vi "TEST_LvMarkdown.vi"() -> ()   [LabVIEW 2021]
uses:
  LvMarkdown/LineBreak/LineBreak.lvclass
  LvMarkdown/Heading/Heading.lvclass
  LvMarkdown/Collection/Collection.lvclass
  LvMarkdown/Paragraph/Paragraph.lvclass
  LvMarkdown/Line/Line.lvclass
  LvMarkdown/HorizontalRule/HorizontalRule.lvclass
  LvMarkdown/Code/Code.lvclass
  LvMarkdown/Bold/Bold.lvclass
  LvMarkdown/Italic/Italic.lvclass
  LvMarkdown/Strikethrough/Strikethrough.lvclass
  LvMarkdown/Blockquote/Blockquote.lvclass
  LvMarkdown/OrderedList/OrderedList.lvclass
  LvMarkdown/UnorderedList/UnorderedList.lvclass
  LvMarkdown/TaskList/TaskList.lvclass
  LvMarkdown/Image/Image.lvclass
  LvMarkdown/Url/Url.lvclass
  LvMarkdown/Link/Link.lvclass
  LvMarkdown/Table/Table.lvclass
  LvMarkdown/Alignment/Alignment.lvclass
  LvMarkdown/FencedCodeBlock/FencedCodeBlock.lvclass
  LvMarkdown/FootnoteReference/FootnoteReference.lvclass
  LvMarkdown/Footnote/Footnote.lvclass
  LvMarkdown/LinkingHeadingId/LinkingHeadingId.lvclass
  LvMarkdown/DefinitionList/DefinitionList.lvclass
  <vilib>/ErrorRing/Error Ring.xnode
  b2edfd4d-23ef-4285-98b5-6188740e71bd.vi
  TEST_LvMarkdownStep.ctl
  LvMarkdown/Alignment/AlignmentEnum.ctl
panel:
  out "String out":string
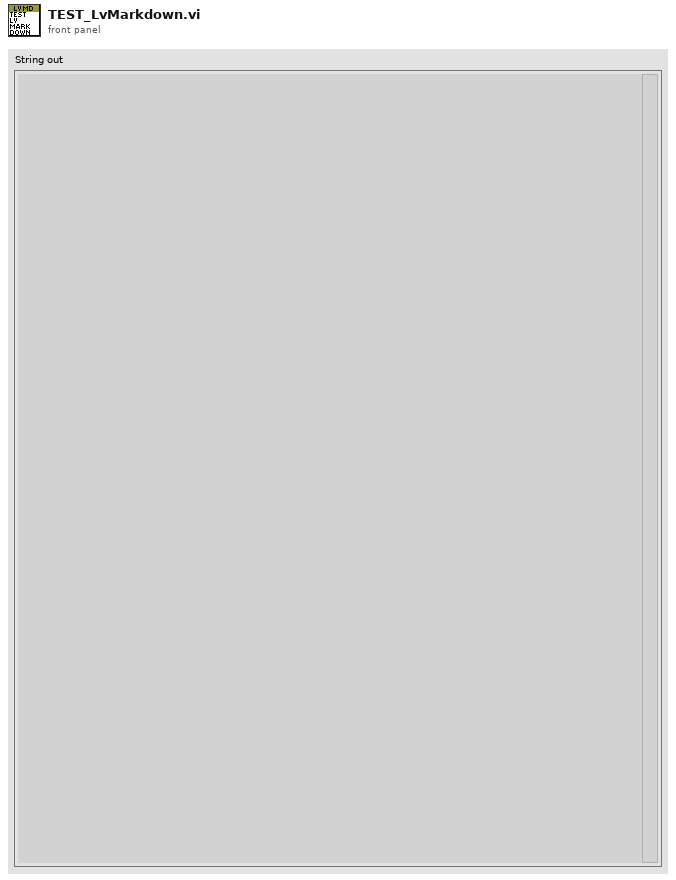
[diagram p1: front panel]
types:
  T1 = enum16{"Level 1", "Level 2", "Level 3", "Level 4", "Level 5", "Level 6"}
  T2 = typedef "TEST_LvMarkdownStep.ctl" = enum16{"Init", "Heading 1", "Paragraph 1", "Heading 2", "Paragraph 2", "Line", "Horizontal Rule", "Emphasis", "Blockquote", "List", "Image", "URL", "Link", "Table", "FencedCodeBlock", "Footnote", "LinkingHeadingId", "DefinitionList", "Exit"}
  T3 = typedef "LvMarkdown.lvlib/Alignment.lvclass/AlignmentEnum.ctl" = enum16{"Left", "Center", "Right"}
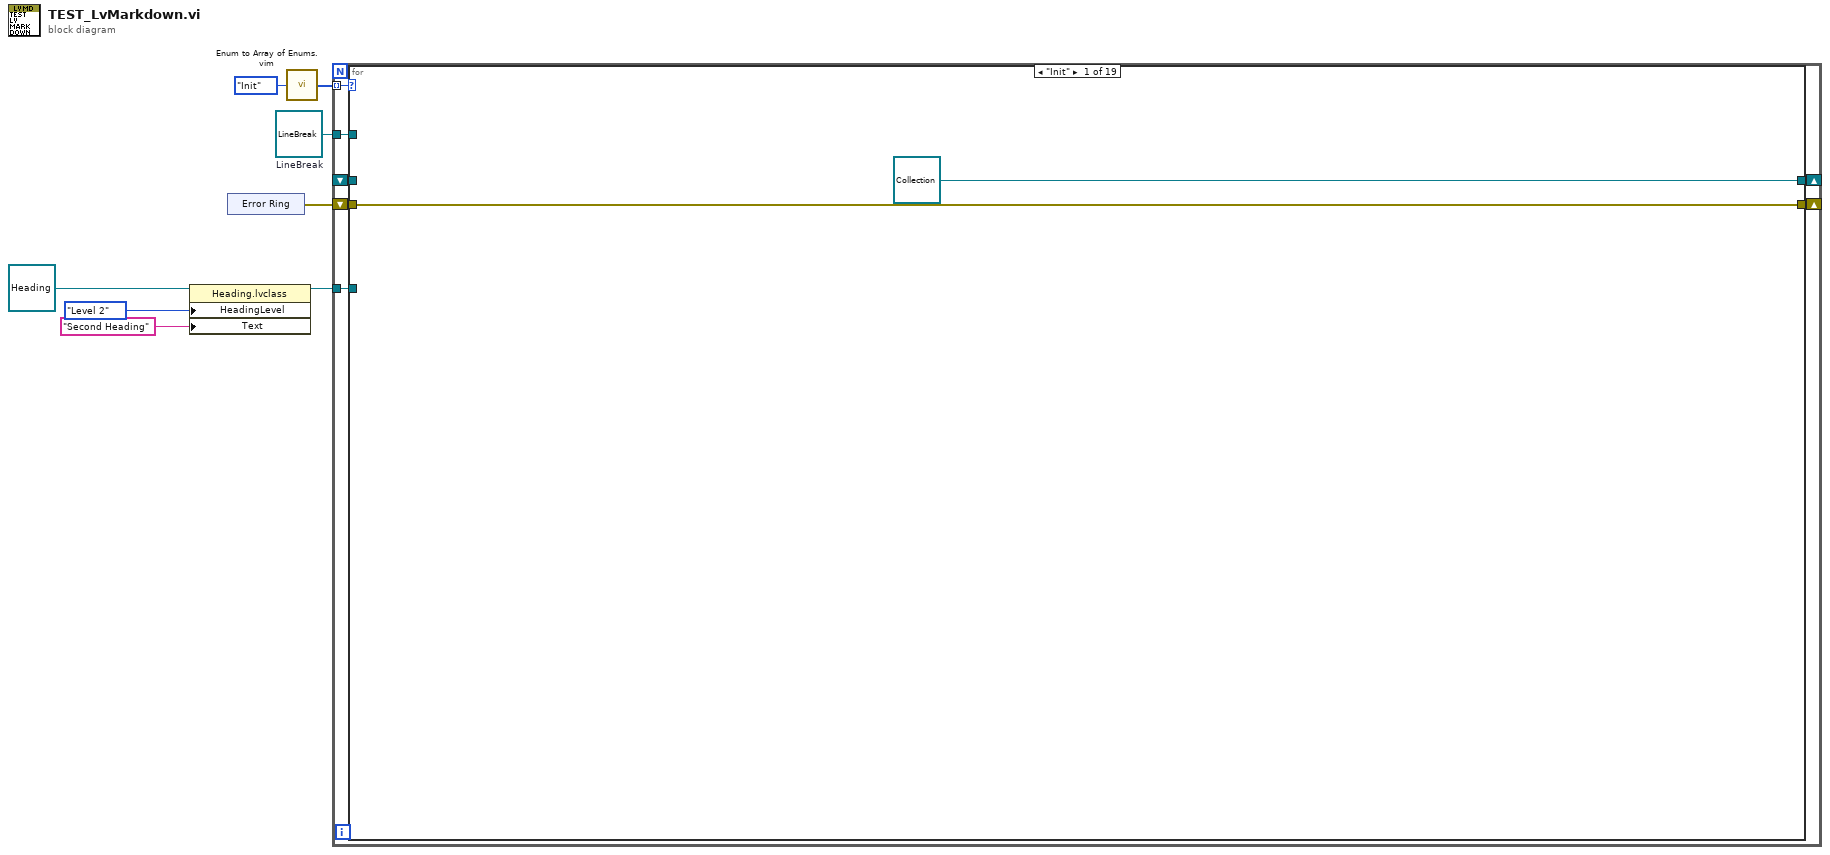
[diagram p0: block diagram]
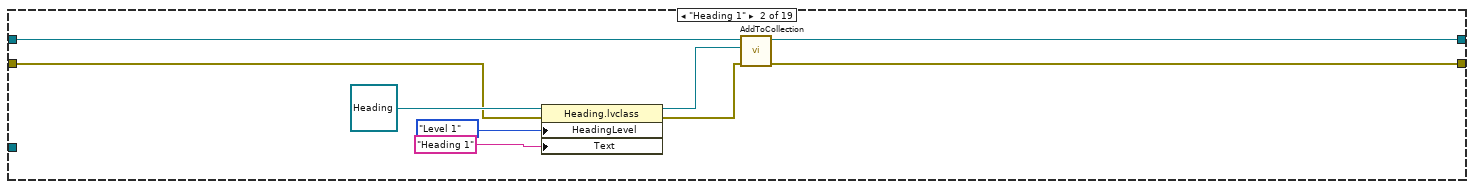
[diagram p2: hidden frame]
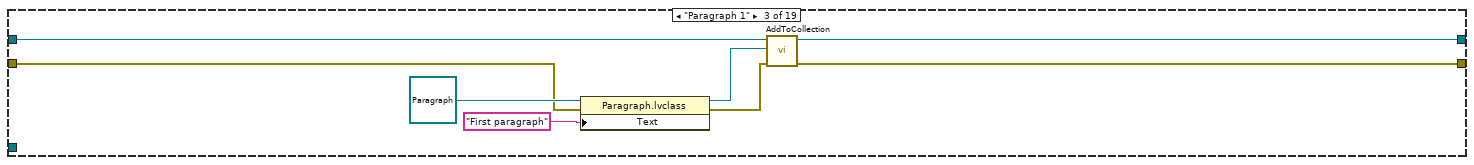
[diagram p3: hidden frame]
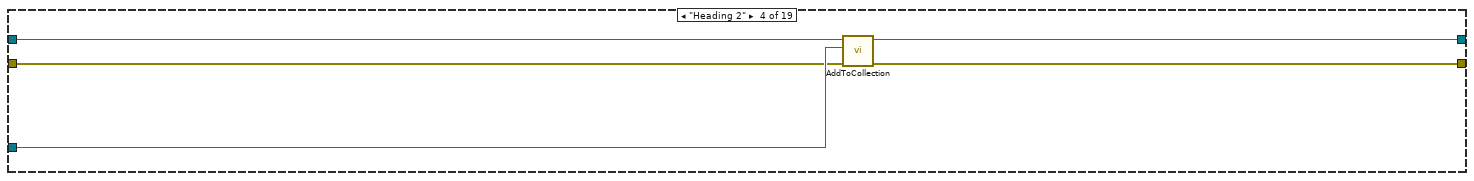
[diagram p4: hidden frame]
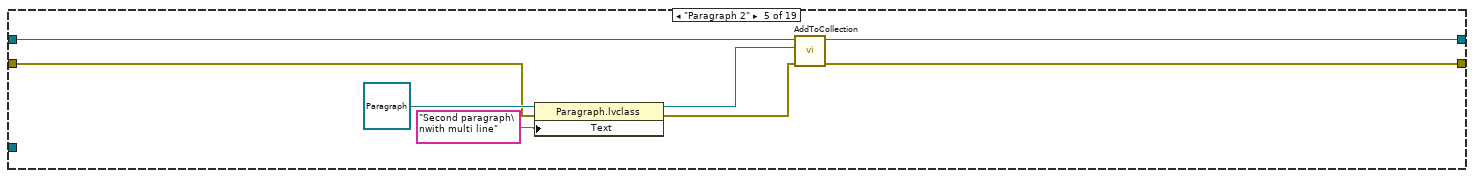
[diagram p5: hidden frame]
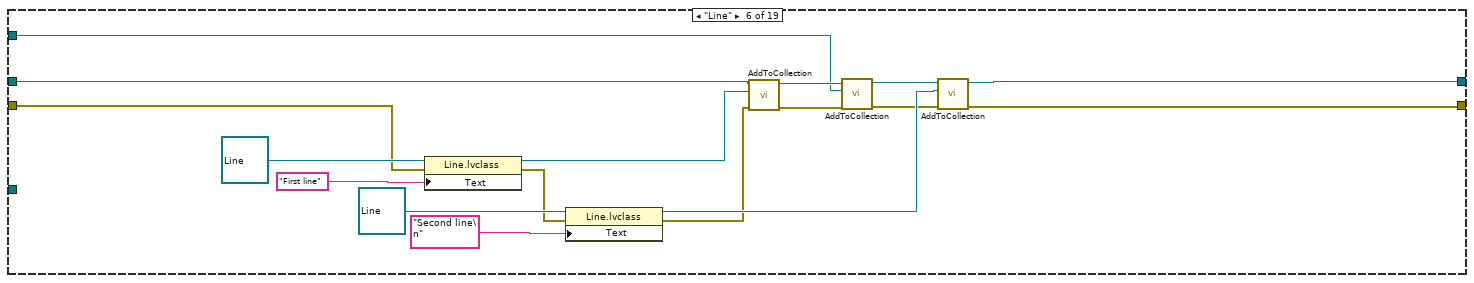
[diagram p6: hidden frame]
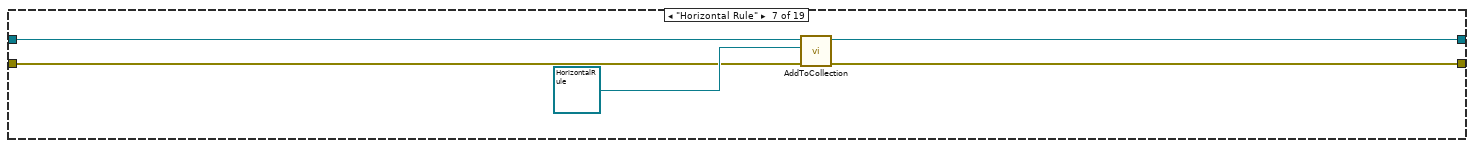
[diagram p7: hidden frame]
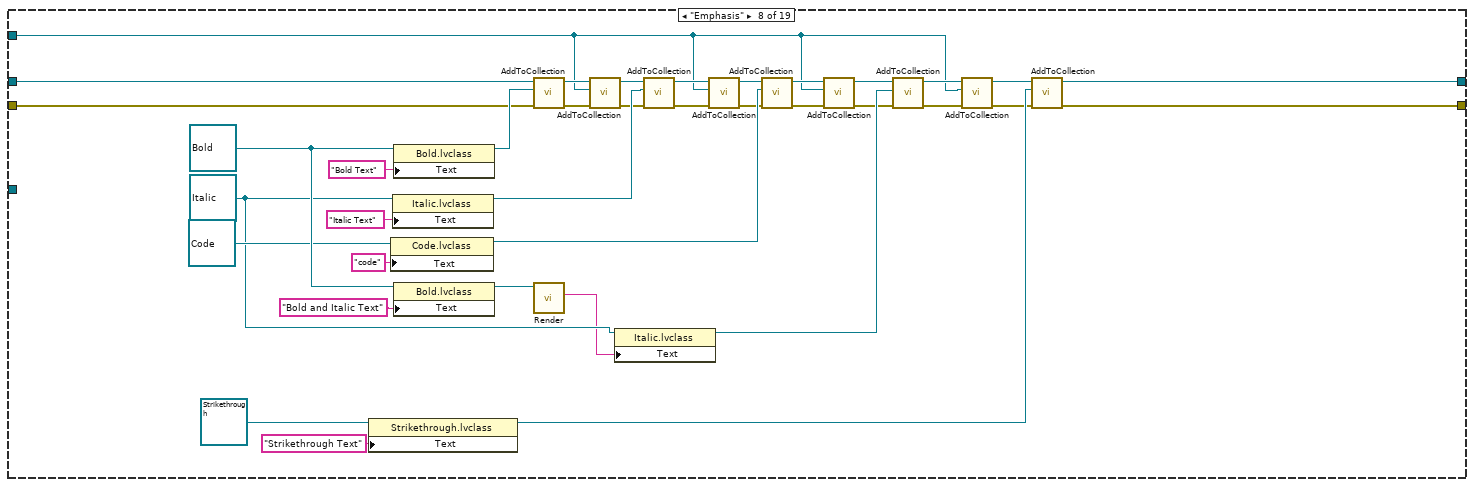
[diagram p8: hidden frame]
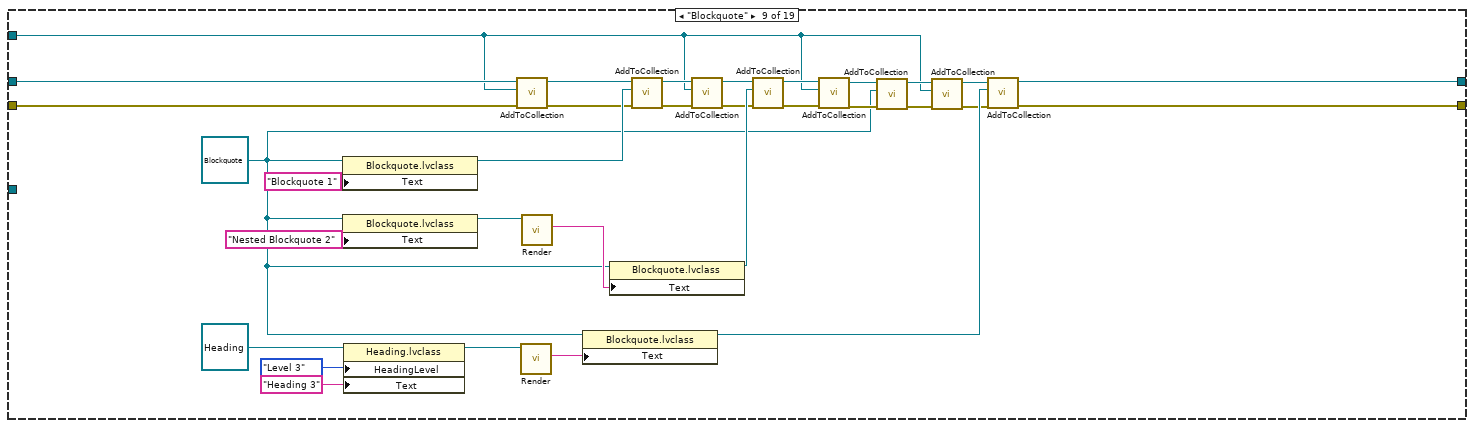
[diagram p9: hidden frame]
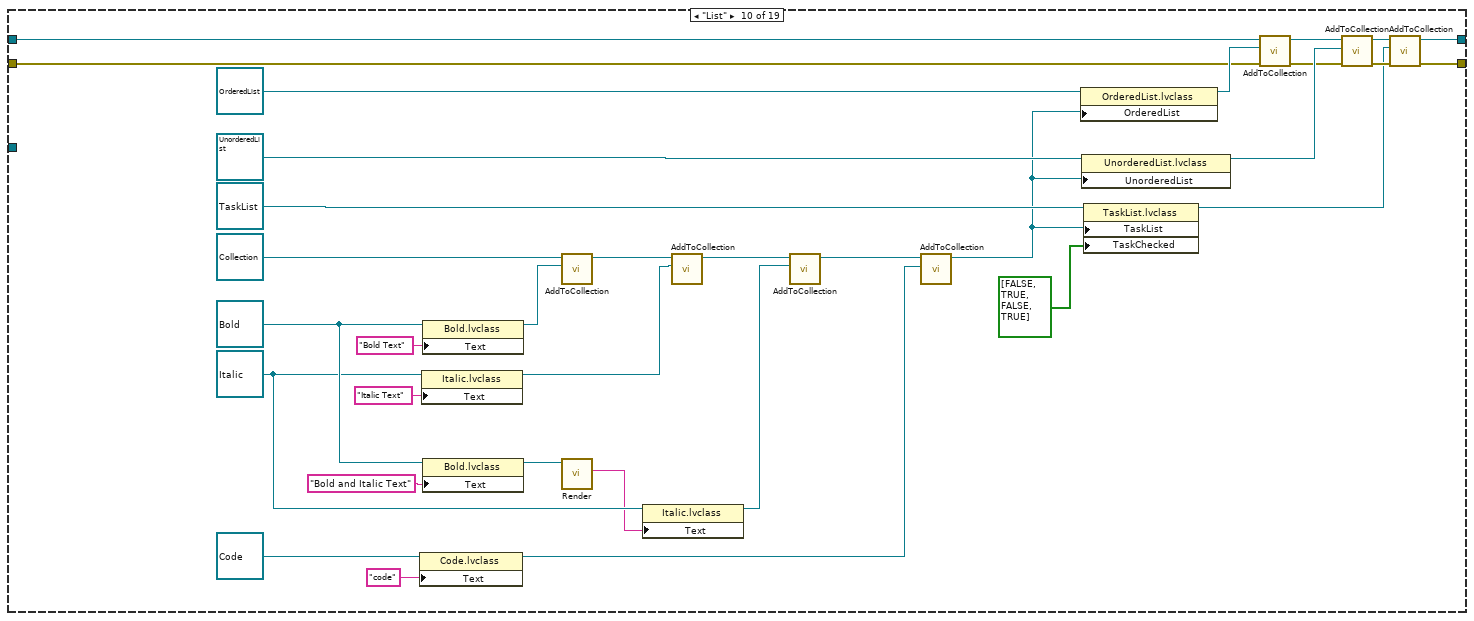
[diagram p10: hidden frame]
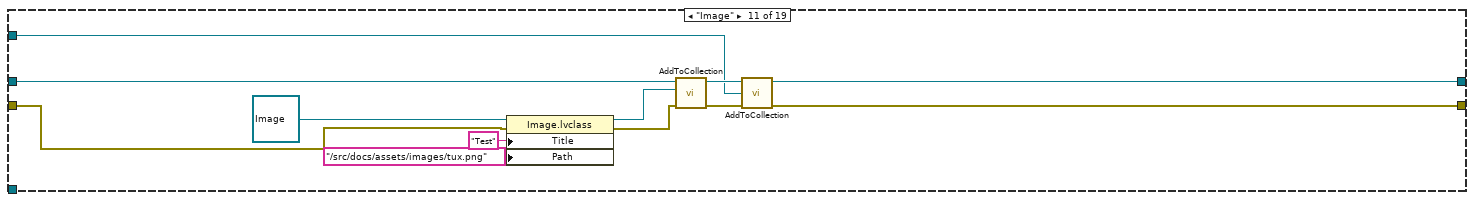
[diagram p11: hidden frame]
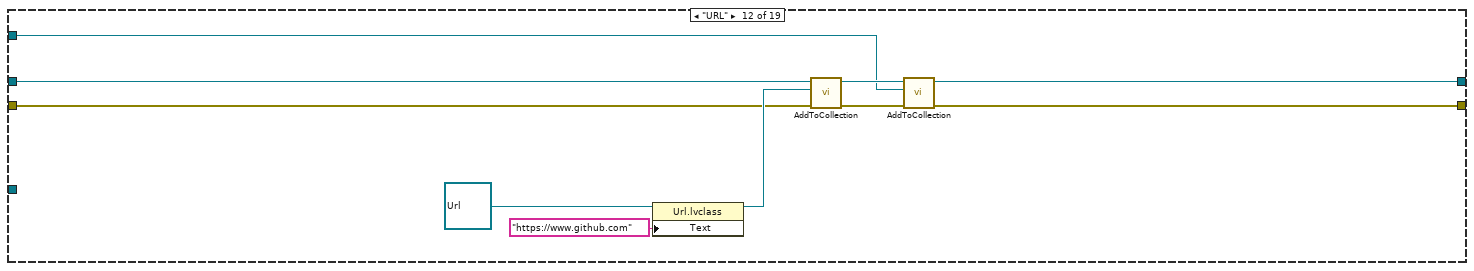
[diagram p12: hidden frame]
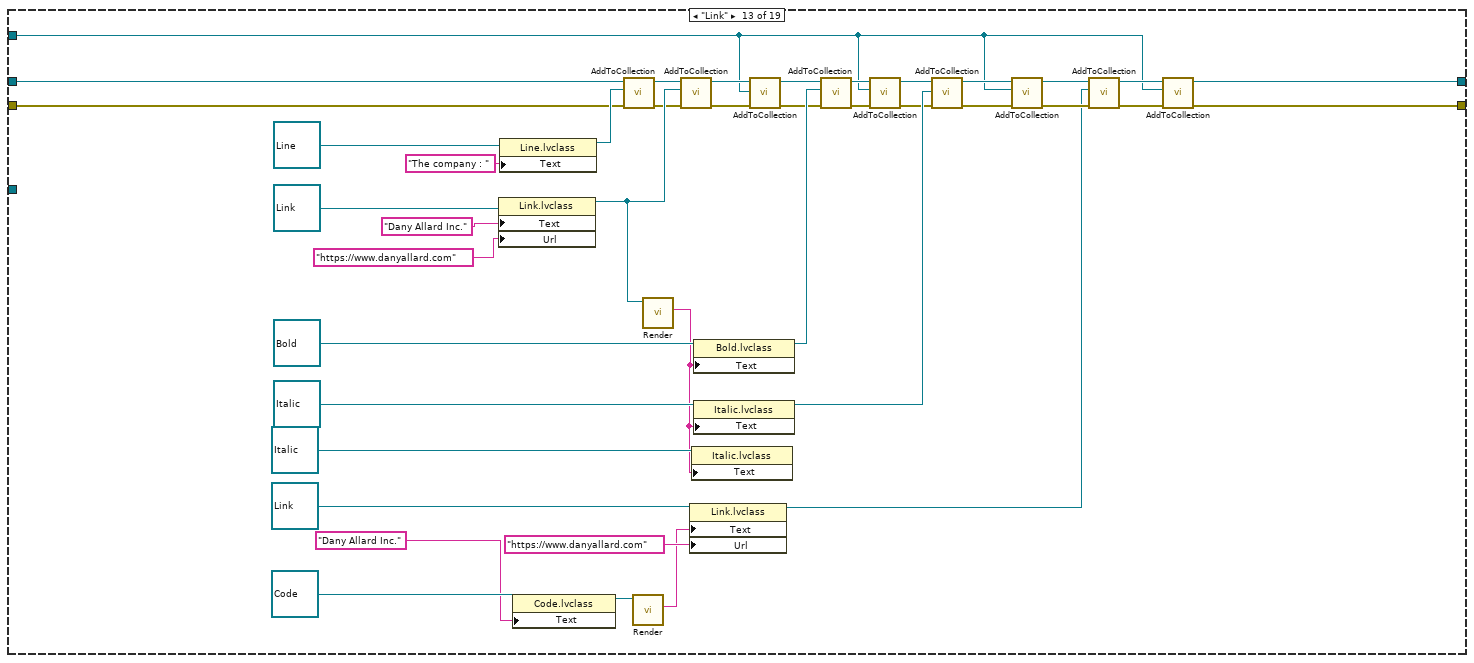
[diagram p13: hidden frame]
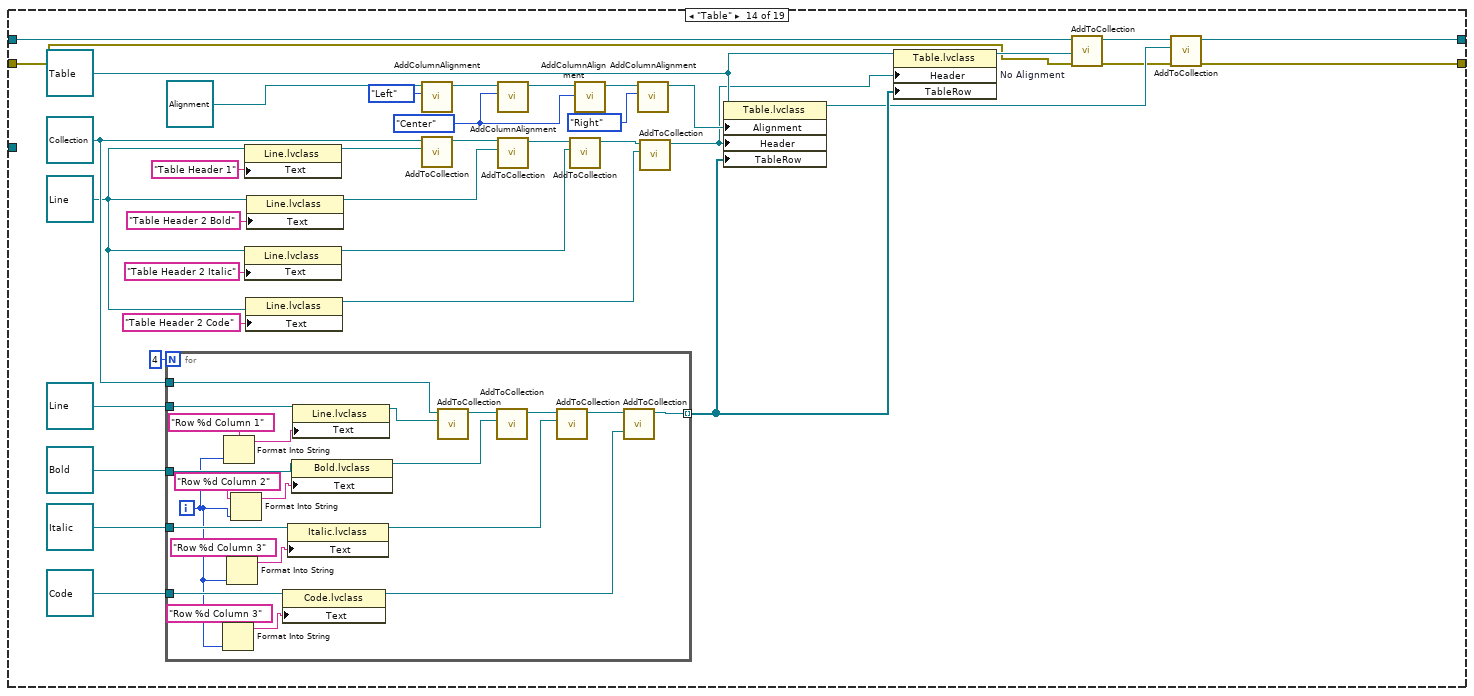
[diagram p14: hidden frame]
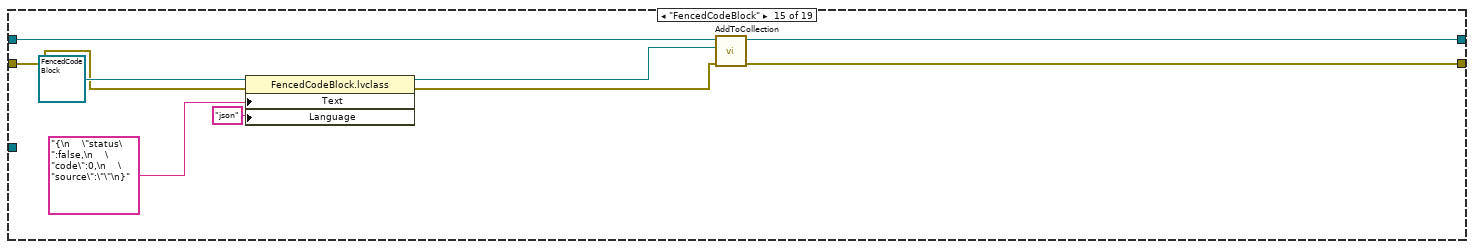
[diagram p15: hidden frame]
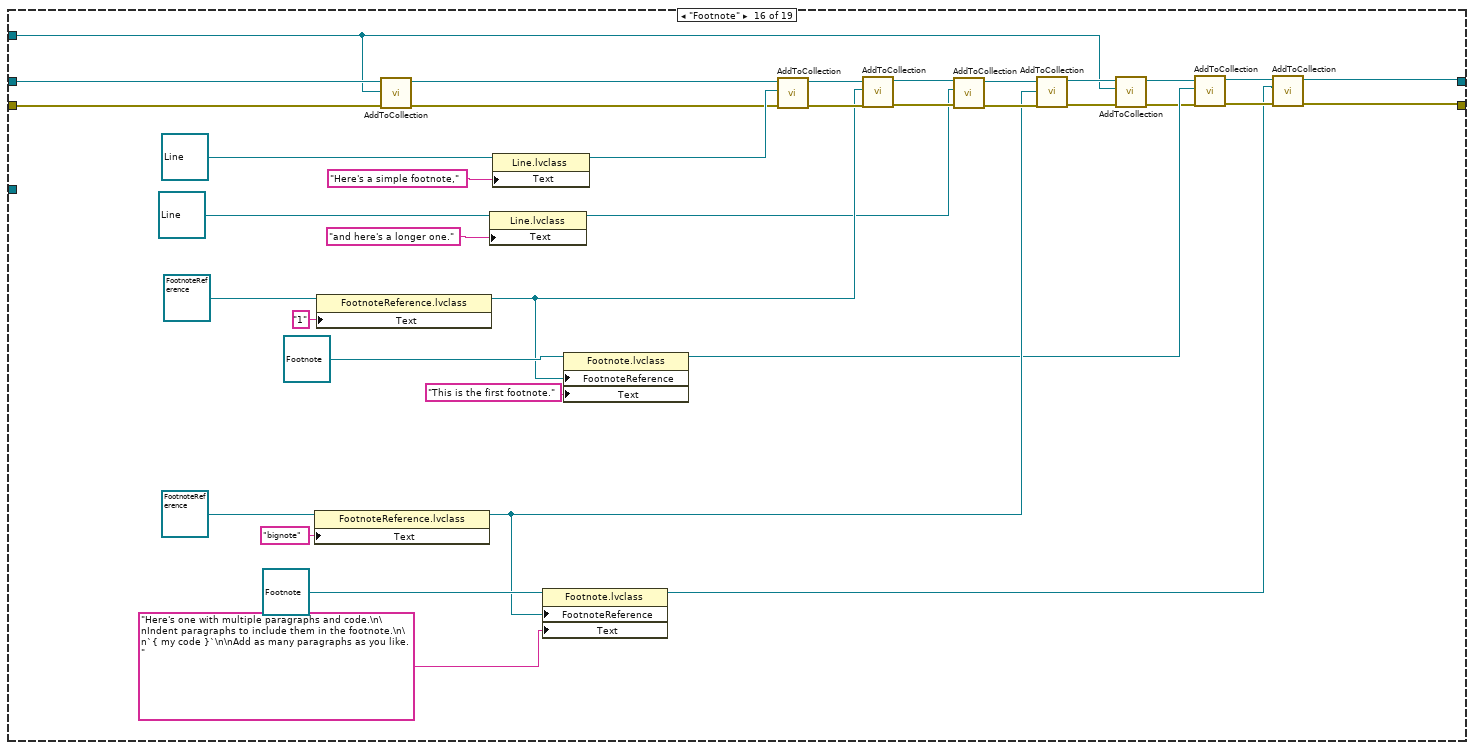
[diagram p16: hidden frame]
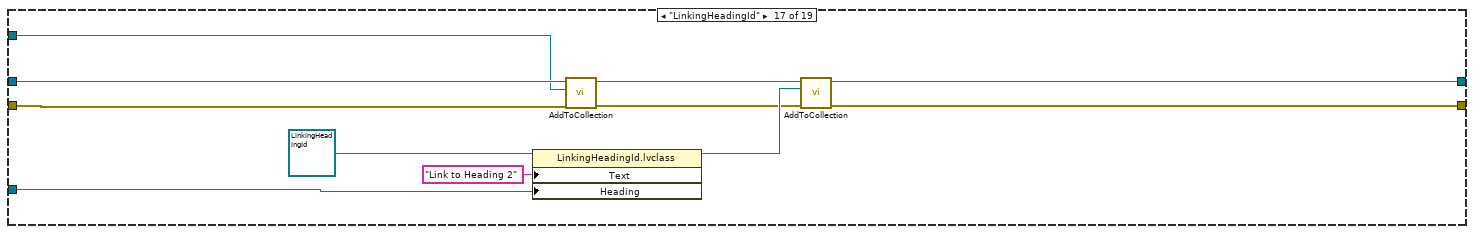
[diagram p17: hidden frame]
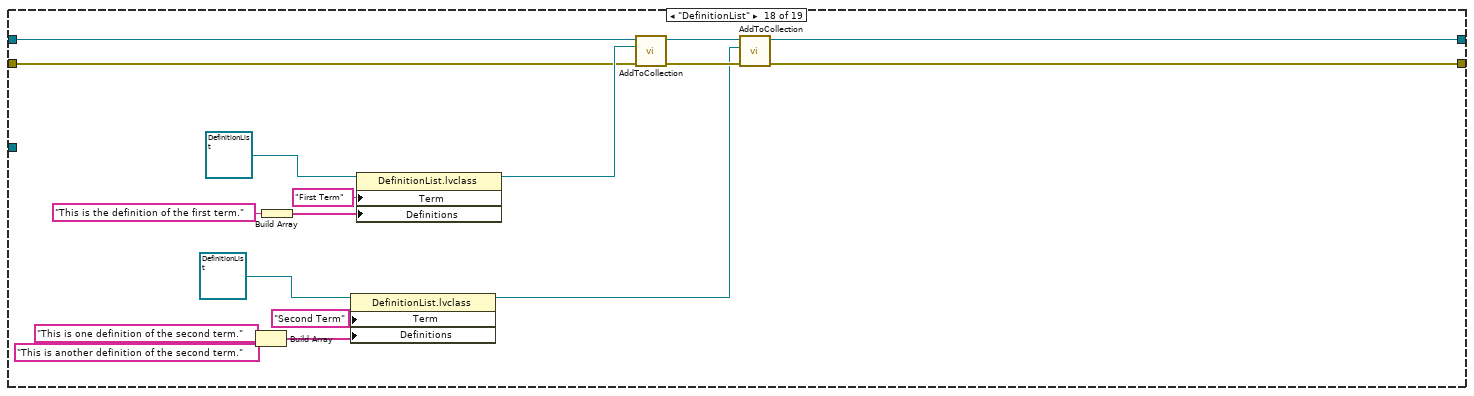
[diagram p18: hidden frame]
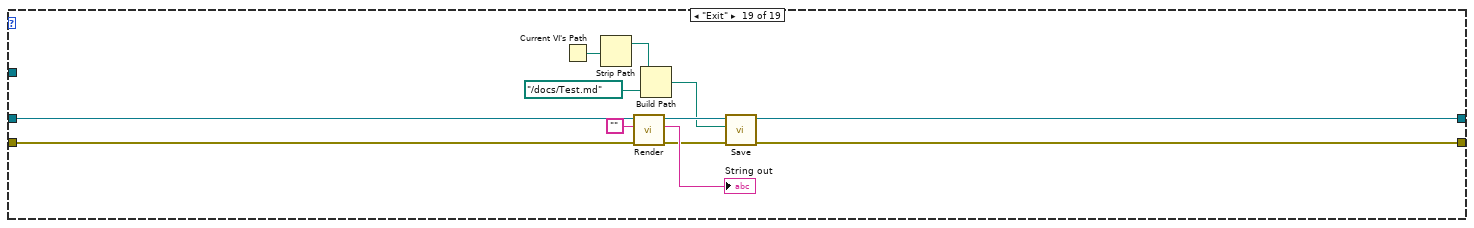
[diagram p19: hidden frame]
diagram:
  w6 = refnum<class "LineBreak.lvclass"> refnum  # LineBreak
  n1 = property class="Heading.lvclass"(reference=refnum<class "Heading.lvclass"> refnum ("Markdown.lvlib:Heading.lvclass"), "HeadingLevel"=T1."Level 2" ("HeadingLevel 2"), "Text"="Second Heading") -> (reference out=w1:refnum<class "Heading.lvclass">)  [unwired: 1 in, 1 out]
  n2 = xnode "Error Ring"() -> ("error out"=w5:errorcluster)
  n3 = call "Enum to Array of Enums.vim"("enum"=TEST_LvMarkdownStep."Init") -> ("array of enums"=w8:T2[])
  n4 = for {
    tunnel: w8 -> [w15] mode=indexing
    shift-right: [w14] -> _
    shift-left: _ -> [w13]
    tunnel: w6 -> [w12]
    shift-right: [w10] -> _
    shift-left: w5 -> [w11]
    tunnel: w1 -> [w9]
    n5 = case shown="\"Init\"" w15 {
      tunnel: [refnum<class "Collection.lvclass"> refnum ("Markdown.lvlib:Collection.lvclass") w22 w31 w37 w45 w58 w69 w76 w123 w141 w177 w188 w197 w241 w298 w322 w346 w353 w371] -> w14
      tunnel: w13 -> [_ w23 w32 w39 w43 w60 w68 w97 w121 w169 w180 w191 w230 w238 w299 w309 w343 w367 w372]
      tunnel: w12 -> [_ _ _ _ _ w54 _ w70 w107 _ w176 w187 w194 _ _ w304 w341 _ _]
      tunnel: w11 -> [w16 w19 w28 w35 w41 w48 w65 w80 w115 w146 w173 w184 w215 w235 w295 w339 w342 w364 w368]
      tunnel: [w16 w18 w27 w38 w40 w51 w66 w77 w116 w143 w172 w185 w195 w236 w294 w323 w344 w354 w369] -> w10
      tunnel: w9 -> [_ _ _ w36 _ _ _ _ _ _ _ _ _ _ _ _ w340 _ _]
      frame "Init" {
      }
      frame "Heading 1" {
        n6 = property class="Heading.lvclass"(reference=refnum<class "Heading.lvclass"> refnum ("Markdown.lvlib:Heading.lvclass"), error in=w19, "HeadingLevel"=T1."Level 1", "Text"="Heading 1") -> (reference out=w21:refnum<class "Heading.lvclass">, error out=w20:errorcluster)
        n7 = call-dynamic "AddToCollection.vi"("error in (no error)"=w20, "IRenderable"=w21, "Collection in"=w23) -> ("error out"=w18:errorcluster, "Collection out"=w22:refnum<class "Collection.lvclass">)  [unwired: 7 in]
      }
      frame "Paragraph 1" {
        n8 = property class="Paragraph.lvclass"(reference=refnum<class "Paragraph.lvclass"> refnum ("Markdown.lvlib:Paragraph.lvclass"), error in=w28, "Text"="First paragraph") -> (reference out=w30:refnum<class "Paragraph.lvclass">, error out=w29:errorcluster)
        n9 = call-dynamic "AddToCollection.vi"("error in (no error)"=w29, "IRenderable"=w30, "Collection in"=w32) -> ("error out"=w27:errorcluster, "Collection out"=w31:refnum<class "Collection.lvclass">)  [unwired: 7 in]
      }
      frame "Heading 2" {
        n10 = call-dynamic "AddToCollection.vi"("error in (no error)"=w35, "IRenderable"=w36, "Collection in"=w39) -> ("error out"=w38:errorcluster, "Collection out"=w37:refnum<class "Collection.lvclass">)  [unwired: 7 in]
      }
      frame "Paragraph 2" {
        n11 = property class="Paragraph.lvclass"(reference=refnum<class "Paragraph.lvclass"> refnum ("Markdown.lvlib:Paragraph.lvclass"), error in=w41, "Text"="Second paragraph\nwith multi line") -> (reference out=w44:refnum<class "Paragraph.lvclass">, error out=w42:errorcluster)
        n12 = call-dynamic "AddToCollection.vi"("error in (no error)"=w42, "IRenderable"=w44, "Collection in"=w43) -> ("error out"=w40:errorcluster, "Collection out"=w45:refnum<class "Collection.lvclass">)  [unwired: 7 in]
      }
      frame "Line" {
        n13 = property class="Line.lvclass"(reference=refnum<class "Line.lvclass"> refnum ("Markdown.lvlib:Line.lvclass"), error in=w48, "Text"="First line") -> (reference out=w57:refnum<class "Line.lvclass">, error out=w50:errorcluster)
        n14 = property class="Line.lvclass"(reference=refnum<class "Line.lvclass"> refnum ("Markdown.lvlib:Line.lvclass"), error in=w50, "Text"="Second line\n") -> (reference out=w56:refnum<class "Line.lvclass">, error out=w49:errorcluster)
        n15 = call-dynamic "AddToCollection.vi"("error in (no error)"=w49, "IRenderable"=w57, "Collection in"=w60) -> ("error out"=w53:errorcluster, "Collection out"=w59:refnum<class "Collection.lvclass">)  [unwired: 7 in]
        n16 = call-dynamic "AddToCollection.vi"("error in (no error)"=w53, "IRenderable"=w54, "Collection in"=w59) -> ("error out"=w52:errorcluster, "Collection out"=w55:refnum<class "Collection.lvclass">)  [unwired: 7 in]
        n17 = call-dynamic "AddToCollection.vi"("error in (no error)"=w52, "IRenderable"=w56, "Collection in"=w55) -> ("error out"=w51:errorcluster, "Collection out"=w58:refnum<class "Collection.lvclass">)  [unwired: 7 in]
      }
      frame "Horizontal Rule" {
        n18 = call-dynamic "AddToCollection.vi"("error in (no error)"=w65, "IRenderable"=refnum<class "HorizontalRule.lvclass"> refnum ("Markdown.lvlib:HorizontalRule.lvclass"), "Collection in"=w68) -> ("error out"=w66:errorcluster, "Collection out"=w69:refnum<class "Collection.lvclass">)  [unwired: 7 in]
      }
      frame "Emphasis" {
        w99 = refnum<class "Italic.lvclass"> refnum ("Markdown.lvlib:Italic.lvclass")
        w104 = refnum<class "Bold.lvclass"> refnum ("Markdown.lvlib:Bold.lvclass")
        n19 = property class="Strikethrough.lvclass"(reference=refnum<class "Strikethrough.lvclass"> refnum ("LvMarkdown.lvlib:Strikethrough.lvclass"), "Text"="Strikethrough Text") -> (reference out=w75:refnum<class "Strikethrough.lvclass">)  [unwired: 1 in, 1 out]
        n20 = property class="Code.lvclass"(reference=refnum<class "Code.lvclass"> refnum ("Markdown.lvlib:Code.lvclass"), "Text"="code") -> (reference out=w90:refnum<class "Code.lvclass">)  [unwired: 1 in, 1 out]
        n21 = property class="Italic.lvclass"(reference=w99, "Text"="Italic Text") -> (reference out=w93:refnum<class "Italic.lvclass">)  [unwired: 1 in, 1 out]
        n22 = property class="Bold.lvclass"(reference=w104, "Text"="Bold Text") -> (reference out=w95:refnum<class "Bold.lvclass">)  [unwired: 1 in, 1 out]
        n23 = property class="Bold.lvclass"(reference=w104, "Text"="Bold and Italic Text") -> (reference out=w103:refnum<class "Bold.lvclass">)  [unwired: 1 in, 1 out]
        n24 = call-dynamic "AddToCollection.vi"("error in (no error)"=w80, "IRenderable"=w95, "Collection in"=w97) -> ("error out"=w86:errorcluster, "Collection out"=w96:refnum<class "Collection.lvclass">)  [unwired: 7 in]
        n25 = call-dynamic "Render.vi"("Bold in"=w103) -> ("String out"=w98:string)  [unwired: 8 in, 2 out]
        n26 = call-dynamic "AddToCollection.vi"("error in (no error)"=w86, "IRenderable"=w70, "Collection in"=w96) -> ("error out"=w85:errorcluster, "Collection out"=w94:refnum<class "Collection.lvclass">)  [unwired: 7 in]
        n27 = property class="Italic.lvclass"(reference=w99, "Text"=w98) -> (reference out=w87:refnum<class "Italic.lvclass">)  [unwired: 1 in, 1 out]
        n28 = call-dynamic "AddToCollection.vi"("error in (no error)"=w85, "IRenderable"=w93, "Collection in"=w94) -> ("error out"=w84:errorcluster, "Collection out"=w92:refnum<class "Collection.lvclass">)  [unwired: 7 in]
        n29 = call-dynamic "AddToCollection.vi"("error in (no error)"=w84, "IRenderable"=w70, "Collection in"=w92) -> ("error out"=w83:errorcluster, "Collection out"=w91:refnum<class "Collection.lvclass">)  [unwired: 7 in]
        n30 = call-dynamic "AddToCollection.vi"("error in (no error)"=w83, "IRenderable"=w90, "Collection in"=w91) -> ("error out"=w82:errorcluster, "Collection out"=w88:refnum<class "Collection.lvclass">)  [unwired: 7 in]
        n31 = call-dynamic "AddToCollection.vi"("error in (no error)"=w82, "IRenderable"=w70, "Collection in"=w88) -> ("error out"=w81:errorcluster, "Collection out"=w89:refnum<class "Collection.lvclass">)  [unwired: 7 in]
        n32 = call-dynamic "AddToCollection.vi"("error in (no error)"=w81, "IRenderable"=w87, "Collection in"=w89) -> ("error out"=w78:errorcluster, "Collection out"=w72:refnum<class "Collection.lvclass">)  [unwired: 7 in]
        n33 = call-dynamic "AddToCollection.vi"("error in (no error)"=w78, "IRenderable"=w70, "Collection in"=w72) -> ("error out"=w73:errorcluster, "Collection out"=w71:refnum<class "Collection.lvclass">)  [unwired: 7 in]
        n34 = call-dynamic "AddToCollection.vi"("error in (no error)"=w73, "IRenderable"=w75, "Collection in"=w71) -> ("error out"=w77:errorcluster, "Collection out"=w76:refnum<class "Collection.lvclass">)  [unwired: 7 in]
      }
      frame "Blockquote" {
        w111 = refnum<class "Blockquote.lvclass"> refnum ("Markdown.lvlib:Blockquote.lvclass")
        n35 = property class="Blockquote.lvclass"(reference=w111, "Text"="Blockquote 1") -> (reference out=w133:refnum<class "Blockquote.lvclass">)  [unwired: 1 in, 1 out]
        n36 = property class="Blockquote.lvclass"(reference=w111, "Text"="Nested Blockquote 2") -> (reference out=w135:refnum<class "Blockquote.lvclass">)  [unwired: 1 in, 1 out]
        n37 = property class="Heading.lvclass"(reference=refnum<class "Heading.lvclass"> refnum ("Markdown.lvlib:Heading.lvclass"), "HeadingLevel"=T1."Level 3", "Text"="Heading 3") -> (reference out=w127:refnum<class "Heading.lvclass">)  [unwired: 1 in, 1 out]
        n38 = call-dynamic "AddToCollection.vi"("error in (no error)"=w115, "IRenderable"=w107, "Collection in"=w121) -> ("error out"=w120:errorcluster, "Collection out"=w122:refnum<class "Collection.lvclass">)  [unwired: 7 in]
        n39 = call-dynamic "Render.vi"("Heading in"=w127) -> ("String out"=w126:string)  [unwired: 8 in, 2 out]
        n40 = call-dynamic "Render.vi"("Blockquote in"=w135) -> ("String out"=w132:string)  [unwired: 8 in, 2 out]
        n41 = property class="Blockquote.lvclass"(reference=w111, "Text"=w126) -> (reference out=w124:refnum<class "Blockquote.lvclass">)  [unwired: 1 in, 1 out]
        n42 = property class="Blockquote.lvclass"(reference=w111, "Text"=w132) -> (reference out=w134:refnum<class "Blockquote.lvclass">)  [unwired: 1 in, 1 out]
        n43 = call-dynamic "AddToCollection.vi"("error in (no error)"=w120, "IRenderable"=w133, "Collection in"=w122) -> ("error out"=w119:errorcluster, "Collection out"=w131:refnum<class "Collection.lvclass">)  [unwired: 7 in]
        n44 = call-dynamic "AddToCollection.vi"("error in (no error)"=w119, "IRenderable"=w107, "Collection in"=w131) -> ("error out"=w118:errorcluster, "Collection out"=w136:refnum<class "Collection.lvclass">)  [unwired: 7 in]
        n45 = call-dynamic "AddToCollection.vi"("error in (no error)"=w118, "IRenderable"=w134, "Collection in"=w136) -> ("error out"=w117:errorcluster, "Collection out"=w125:refnum<class "Collection.lvclass">)  [unwired: 7 in]
        n46 = call-dynamic "AddToCollection.vi"("error in (no error)"=w117, "IRenderable"=w107, "Collection in"=w125) -> ("error out"=w114:errorcluster, "Collection out"=w113:refnum<class "Collection.lvclass">)  [unwired: 7 in]
        n47 = call-dynamic "AddToCollection.vi"("error in (no error)"=w114, "IRenderable"=w111, "Collection in"=w113) -> ("error out"=w112:errorcluster, "Collection out"=w109:refnum<class "Collection.lvclass">)  [unwired: 7 in]
        n48 = call-dynamic "AddToCollection.vi"("error in (no error)"=w112, "IRenderable"=w107, "Collection in"=w109) -> ("error out"=w110:errorcluster, "Collection out"=w108:refnum<class "Collection.lvclass">)  [unwired: 7 in]
        n49 = call-dynamic "AddToCollection.vi"("error in (no error)"=w110, "IRenderable"=w124, "Collection in"=w108) -> ("error out"=w116:errorcluster, "Collection out"=w123:refnum<class "Collection.lvclass">)  [unwired: 7 in]
      }
      frame "List" {
        w161 = refnum<class "Italic.lvclass"> refnum ("Markdown.lvlib:Italic.lvclass")
        w166 = refnum<class "Bold.lvclass"> refnum ("Markdown.lvlib:Bold.lvclass")
        n50 = property class="Code.lvclass"(reference=refnum<class "Code.lvclass"> refnum ("Markdown.lvlib:Code.lvclass"), "Text"="code") -> (reference out=w150:refnum<class "Code.lvclass">)  [unwired: 1 in, 1 out]
        n51 = property class="Italic.lvclass"(reference=w161, "Text"="Italic Text") -> (reference out=w158:refnum<class "Italic.lvclass">)  [unwired: 1 in, 1 out]
        n52 = property class="Bold.lvclass"(reference=w166, "Text"="Bold Text") -> (reference out=w159:refnum<class "Bold.lvclass">)  [unwired: 1 in, 1 out]
        n53 = property class="Bold.lvclass"(reference=w166, "Text"="Bold and Italic Text") -> (reference out=w165:refnum<class "Bold.lvclass">)  [unwired: 1 in, 1 out]
        n54 = call-dynamic "AddToCollection.vi"("IRenderable"=w159, "Collection in"=refnum<class "Collection.lvclass"> refnum) -> ("Collection out"=w154:refnum<class "Collection.lvclass">)  [unwired: 8 in, 1 out]
        n55 = call-dynamic "Render.vi"("Bold in"=w165) -> ("String out"=w160:string)  [unwired: 8 in, 2 out]
        n56 = property class="Italic.lvclass"(reference=w161, "Text"=w160) -> (reference out=w149:refnum<class "Italic.lvclass">)  [unwired: 1 in, 1 out]
        n57 = call-dynamic "AddToCollection.vi"("IRenderable"=w158, "Collection in"=w154) -> ("Collection out"=w157:refnum<class "Collection.lvclass">)  [unwired: 8 in, 1 out]
        n58 = call-dynamic "AddToCollection.vi"("IRenderable"=w149, "Collection in"=w157) -> ("Collection out"=w156:refnum<class "Collection.lvclass">)  [unwired: 8 in, 1 out]
        n59 = call-dynamic "AddToCollection.vi"("IRenderable"=w150, "Collection in"=w156) -> ("Collection out"=w144:refnum<class "Collection.lvclass">)  [unwired: 8 in, 1 out]
        n60 = property class="OrderedList.lvclass"(reference=refnum<class "OrderedList.lvclass"> refnum ("Markdown.lvlib:OrderedList.lvclass"), "OrderedList"=w144) -> (reference out=w153:refnum<class "OrderedList.lvclass">)  [unwired: 1 in, 1 out]
        n61 = property class="UnorderedList.lvclass"(reference=refnum<class "UnorderedList.lvclass"> refnum ("Markdown.lvlib:UnorderedList.lvclass"), "UnorderedList"=w144) -> (reference out=w151:refnum<class "UnorderedList.lvclass">)  [unwired: 1 in, 1 out]
        n62 = property class="TaskList.lvclass"(reference=refnum<class "TaskList.lvclass"> refnum ("LvMarkdown.lvlib:TaskList.lvclass"), "TaskList"=w144, "TaskChecked"=bool[] [FALSE, TRUE, FALSE, TRUE]) -> (reference out=w140:refnum<class "TaskList.lvclass">)  [unwired: 1 in, 1 out]
        n63 = call-dynamic "AddToCollection.vi"("error in (no error)"=w146, "IRenderable"=w153, "Collection in"=w169) -> ("error out"=w148:errorcluster, "Collection out"=w152:refnum<class "Collection.lvclass">)  [unwired: 7 in]
        n64 = call-dynamic "AddToCollection.vi"("error in (no error)"=w148, "IRenderable"=w151, "Collection in"=w152) -> ("error out"=w147:errorcluster, "Collection out"=w142:refnum<class "Collection.lvclass">)  [unwired: 7 in]
        n65 = call-dynamic "AddToCollection.vi"("error in (no error)"=w147, "IRenderable"=w140, "Collection in"=w142) -> ("error out"=w143:errorcluster, "Collection out"=w141:refnum<class "Collection.lvclass">)  [unwired: 7 in]
      }
      frame "Image" {
        n66 = property class="Image.lvclass"(reference=refnum<class "Image.lvclass"> refnum ("Markdown.lvlib:Image.lvclass"), error in=w173, "Title"="Test", "Path"="/src/docs/assets/images/tux.png") -> (reference out=w181:refnum<class "Image.lvclass">, error out=w175:errorcluster)
        n67 = call-dynamic "AddToCollection.vi"("error in (no error)"=w175, "IRenderable"=w181, "Collection in"=w180) -> ("error out"=w174:errorcluster, "Collection out"=w179:refnum<class "Collection.lvclass">)  [unwired: 7 in]
        n68 = call-dynamic "AddToCollection.vi"("error in (no error)"=w174, "IRenderable"=w176, "Collection in"=w179) -> ("error out"=w172:errorcluster, "Collection out"=w177:refnum<class "Collection.lvclass">)  [unwired: 7 in]
      }
      frame "URL" {
        n69 = property class="Url.lvclass"(reference=refnum<class "Url.lvclass"> refnum ("Markdown.lvlib:Url.lvclass"), "Text"="https://www.github.com") -> (reference out=w189:refnum<class "Url.lvclass">)  [unwired: 1 in, 1 out]
        n70 = call-dynamic "AddToCollection.vi"("error in (no error)"=w184, "IRenderable"=w189, "Collection in"=w191) -> ("error out"=w186:errorcluster, "Collection out"=w190:refnum<class "Collection.lvclass">)  [unwired: 7 in]
        n71 = call-dynamic "AddToCollection.vi"("error in (no error)"=w186, "IRenderable"=w187, "Collection in"=w190) -> ("error out"=w185:errorcluster, "Collection out"=w188:refnum<class "Collection.lvclass">)  [unwired: 7 in]
      }
      frame "Link" {
        n72 = property class="Link.lvclass"(reference=refnum<class "Link.lvclass"> refnum ("Markdown.lvlib:Link.lvclass"), "Text"="Dany Allard Inc.", "Url"="https://www.danyallard.com" ("Text")) -> (reference out=w224:refnum<class "Link.lvclass">)  [unwired: 1 in, 1 out]
        n73 = property class="Line.lvclass"(reference=refnum<class "Line.lvclass"> refnum ("Markdown.lvlib:Line.lvclass"), "Text"="The company : ") -> (reference out=w229:refnum<class "Line.lvclass">)  [unwired: 1 in, 1 out]
        n74 = property class="Code.lvclass"(reference=refnum<class "Code.lvclass"> refnum ("Markdown.lvlib:Code.lvclass"), "Text"="Dany Allard Inc.") -> (reference out=w201:refnum<class "Code.lvclass">)  [unwired: 1 in, 1 out]
        n75 = call-dynamic "AddToCollection.vi"("error in (no error)"=w215, "IRenderable"=w229, "Collection in"=w230) -> ("error out"=w214:errorcluster, "Collection out"=w228:refnum<class "Collection.lvclass">)  [unwired: 7 in]
        n76 = call-dynamic "Render.vi"("Bold in"=w201) -> ("String out"=w200:string)  [unwired: 8 in, 2 out]
        n77 = call-dynamic "Render.vi"("Link in"=w224) -> ("String out"=w206:string)  [unwired: 8 in, 2 out]
        n78 = call-dynamic "AddToCollection.vi"("error in (no error)"=w214, "IRenderable"=w224, "Collection in"=w228) -> ("error out"=w213:errorcluster, "Collection out"=w223:refnum<class "Collection.lvclass">)  [unwired: 7 in]
        n79 = property class="Link.lvclass"(reference=refnum<class "Link.lvclass"> refnum ("Markdown.lvlib:Link.lvclass"), "Text"=w200, "Url"="https://www.danyallard.com" ("Text")) -> (reference out=w199:refnum<class "Link.lvclass">)  [unwired: 1 in, 1 out]
        n80 = property class="Italic.lvclass"(reference=refnum<class "Italic.lvclass"> refnum ("Markdown.lvlib:Italic.lvclass"), "Text"=w206) -> ()  [unwired: 1 in, 2 out]
        n81 = property class="Bold.lvclass"(reference=refnum<class "Bold.lvclass"> refnum ("Markdown.lvlib:Bold.lvclass"), "Text"=w206) -> (reference out=w219:refnum<class "Bold.lvclass">)  [unwired: 1 in, 1 out]
        n82 = property class="Italic.lvclass"(reference=refnum<class "Italic.lvclass"> refnum ("Markdown.lvlib:Italic.lvclass"), "Text"=w206) -> (reference out=w218:refnum<class "Italic.lvclass">)  [unwired: 1 in, 1 out]
        n83 = call-dynamic "AddToCollection.vi"("error in (no error)"=w213, "IRenderable"=w194, "Collection in"=w223) -> ("error out"=w212:errorcluster, "Collection out"=w222:refnum<class "Collection.lvclass">)  [unwired: 7 in]
        n84 = call-dynamic "AddToCollection.vi"("error in (no error)"=w212, "IRenderable"=w219, "Collection in"=w222) -> ("error out"=w211:errorcluster, "Collection out"=w221:refnum<class "Collection.lvclass">)  [unwired: 7 in]
        n85 = call-dynamic "AddToCollection.vi"("error in (no error)"=w211, "IRenderable"=w194, "Collection in"=w221) -> ("error out"=w210:errorcluster, "Collection out"=w220:refnum<class "Collection.lvclass">)  [unwired: 7 in]
        n86 = call-dynamic "AddToCollection.vi"("error in (no error)"=w210, "IRenderable"=w218, "Collection in"=w220) -> ("error out"=w209:errorcluster, "Collection out"=w217:refnum<class "Collection.lvclass">)  [unwired: 7 in]
        n87 = call-dynamic "AddToCollection.vi"("error in (no error)"=w209, "IRenderable"=w194, "Collection in"=w217) -> ("error out"=w208:errorcluster, "Collection out"=w216:refnum<class "Collection.lvclass">)  [unwired: 7 in]
        n88 = call-dynamic "AddToCollection.vi"("error in (no error)"=w208, "IRenderable"=w199, "Collection in"=w216) -> ("error out"=w196:errorcluster, "Collection out"=w198:refnum<class "Collection.lvclass">)  [unwired: 7 in]
        n89 = call-dynamic "AddToCollection.vi"("error in (no error)"=w196, "IRenderable"=w194, "Collection in"=w198) -> ("error out"=w195:errorcluster, "Collection out"=w197:refnum<class "Collection.lvclass">)  [unwired: 7 in]
      }
      frame "Table" {
        w248 = AlignmentEnum."Center" ("Alignment")
        w266 = refnum<class "Collection.lvclass"> refnum ("Collection in")
        w258 = refnum<class "Line.lvclass"> refnum ("Markdown.lvlib:Line.lvclass")
        w245 = refnum<class "Table.lvclass"> refnum ("LvMarkdown.lvlib:Table.lvclass")
        n90 = for {
          N: 4 -> [_]
          tunnel: refnum<class "Bold.lvclass"> refnum ("Markdown.lvlib:Bold.lvclass") -> [w289]
          tunnel: w266 -> [w291]
          tunnel: [w276] -> w244 mode=indexing
          tunnel: refnum<class "Line.lvclass"> refnum ("Markdown.lvlib:Line.lvclass") -> [w284]
          tunnel: refnum<class "Italic.lvclass"> refnum ("Markdown.lvlib:Italic.lvclass") -> [w282]
          tunnel: refnum<class "Code.lvclass"> refnum ("Markdown.lvlib:Code.lvclass") -> [w279]
          i -> [w274]
          n91 = Format Into String(format string="Row %d Column 3" ("Text"), w274) -> (resulting string=w278:string)  [unwired: 2 in, 1 out]
          n92 = Format Into String(format string="Row %d Column 1" ("Text"), w274) -> (resulting string=w288:string)  [unwired: 2 in, 1 out]
          n93 = Format Into String(format string="Row %d Column 3" ("Text"), w274) -> (resulting string=w283:string)  [unwired: 2 in, 1 out]
          n94 = Format Into String(format string="Row %d Column 2" ("Text"), w274) -> (resulting string=w287:string)  [unwired: 2 in, 1 out]
          n95 = property class="Code.lvclass"(reference=w279, "Text"=w278) -> (reference out=w275:refnum<class "Code.lvclass">)  [unwired: 1 in, 1 out]
          n96 = property class="Italic.lvclass"(reference=w282, "Text"=w283) -> (reference out=w280:refnum<class "Italic.lvclass">)  [unwired: 1 in, 1 out]
          n97 = property class="Bold.lvclass"(reference=w289, "Text"=w287) -> (reference out=w290:refnum<class "Bold.lvclass">)  [unwired: 1 in, 1 out]
          n98 = property class="Line.lvclass"(reference=w284, "Text"=w288) -> (reference out=w292:refnum<class "Line.lvclass">)  [unwired: 1 in, 1 out]
          n99 = call-dynamic "AddToCollection.vi"("IRenderable"=w292, "Collection in"=w291) -> ("Collection out"=w293:refnum<class "Collection.lvclass">)  [unwired: 8 in, 1 out]
          n100 = call-dynamic "AddToCollection.vi"("IRenderable"=w290, "Collection in"=w293) -> ("Collection out"=w281:refnum<class "Collection.lvclass">)  [unwired: 8 in, 1 out]
          n101 = call-dynamic "AddToCollection.vi"("IRenderable"=w280, "Collection in"=w281) -> ("Collection out"=w277:refnum<class "Collection.lvclass">)  [unwired: 8 in, 1 out]
          n102 = call-dynamic "AddToCollection.vi"("IRenderable"=w275, "Collection in"=w277) -> ("Collection out"=w276:refnum<class "Collection.lvclass">)  [unwired: 8 in, 1 out]
        }
        n103 = property class="Line.lvclass"(reference=w258, "Text"="Table Header 1") -> (reference out=w268:refnum<class "Line.lvclass">)  [unwired: 1 in, 1 out]
        n104 = property class="Line.lvclass"(reference=w258, "Text"="Table Header 2 Italic") -> (reference out=w255:refnum<class "Line.lvclass">)  [unwired: 1 in, 1 out]
        n105 = property class="Line.lvclass"(reference=w258, "Text"="Table Header 2 Code") -> (reference out=w254:refnum<class "Line.lvclass">)  [unwired: 1 in, 1 out]
        n106 = property class="Line.lvclass"(reference=w258, "Text"="Table Header 2 Bold") -> (reference out=w269:refnum<class "Line.lvclass">)  [unwired: 1 in, 1 out]
        n107 = call "AddColumnAlignment.vi"("Alignment"=AlignmentEnum."Left", "Alignment in"=refnum<class "Alignment.lvclass"> refnum ("LvMarkdown.lvlib:Alignment.lvclass")) -> ("Alignment out"=w253:refnum<class "Alignment.lvclass">)  [unwired: 8 in, 1 out]
        n108 = call-dynamic "AddToCollection.vi"("IRenderable"=w268, "Collection in"=w266) -> ("Collection out"=w267:refnum<class "Collection.lvclass">)  [unwired: 8 in, 1 out]
        n109 = call "AddColumnAlignment.vi"("Alignment"=w248, "Alignment in"=w253) -> ("Alignment out"=w252:refnum<class "Alignment.lvclass">)  [unwired: 8 in, 1 out]
        n110 = call-dynamic "AddToCollection.vi"("IRenderable"=w269, "Collection in"=w267) -> ("Collection out"=w256:refnum<class "Collection.lvclass">)  [unwired: 8 in, 1 out]
        n111 = call-dynamic "AddToCollection.vi"("IRenderable"=w255, "Collection in"=w256) -> ("Collection out"=w257:refnum<class "Collection.lvclass">)  [unwired: 8 in, 1 out]
        n112 = call "AddColumnAlignment.vi"("Alignment"=w248, "Alignment in"=w252) -> ("Alignment out"=w251:refnum<class "Alignment.lvclass">)  [unwired: 8 in, 1 out]
        n113 = call "AddColumnAlignment.vi"("Alignment"=AlignmentEnum."Right", "Alignment in"=w251) -> ("Alignment out"=w250:refnum<class "Alignment.lvclass">)  [unwired: 8 in, 1 out]
        n114 = call-dynamic "AddToCollection.vi"("IRenderable"=w254, "Collection in"=w257) -> ("Collection out"=w243:refnum<class "Collection.lvclass">)  [unwired: 8 in, 1 out]
        n115 = property class="Table.lvclass"(reference=w245, "Alignment"=w250, "Header"=w243, "TableRow"=w244) -> (reference out=w240:refnum<class "Table.lvclass">)  [unwired: 1 in, 1 out]
        n116 = property on="No Alignment" class="Table.lvclass"(reference=w245, "Header"=w243, "TableRow"=w244) -> (reference out=w239:refnum<class "Table.lvclass">)  [unwired: 1 in, 1 out]
        n117 = call-dynamic "AddToCollection.vi"("error in (no error)"=w235, "IRenderable"=w239, "Collection in"=w238) -> ("error out"=w237:errorcluster, "Collection out"=w242:refnum<class "Collection.lvclass">)  [unwired: 7 in]
        n118 = call-dynamic "AddToCollection.vi"("error in (no error)"=w237, "IRenderable"=w240, "Collection in"=w242) -> ("error out"=w236:errorcluster, "Collection out"=w241:refnum<class "Collection.lvclass">)  [unwired: 7 in]
      }
      frame "FencedCodeBlock" {
        n119 = property class="FencedCodeBlock.lvclass"(reference=refnum<class "FencedCodeBlock.lvclass"> refnum ("LvMarkdown.lvlib:FencedCodeBlock.lvclass"), error in=w295, "Text"="{\n    \"status\":false,\n    \"code\":0,\n    \"source\":\"\"\n}", "Language"="json") -> (reference out=w297:refnum<class "FencedCodeBlock.lvclass">, error out=w296:errorcluster)
        n120 = call-dynamic "AddToCollection.vi"("error in (no error)"=w296, "IRenderable"=w297, "Collection in"=w299) -> ("error out"=w294:errorcluster, "Collection out"=w298:refnum<class "Collection.lvclass">)  [unwired: 7 in]
      }
      frame "Footnote" {
        n121 = property class="FootnoteReference.lvclass"(reference=refnum<class "FootnoteReference.lvclass"> refnum ("LvMarkdown.lvlib:FootnoteReference.lvclass"), "Text"="bignote") -> (reference out=w314:refnum<class "FootnoteReference.lvclass">)  [unwired: 1 in, 1 out]
        n122 = property class="FootnoteReference.lvclass"(reference=refnum<class "FootnoteReference.lvclass"> refnum ("LvMarkdown.lvlib:FootnoteReference.lvclass"), "Text"="1") -> (reference out=w321:refnum<class "FootnoteReference.lvclass">)  [unwired: 1 in, 1 out]
        n123 = call-dynamic "AddToCollection.vi"("error in (no error)"=w339, "IRenderable"=w304, "Collection in"=w309) -> ("error out"=w310:errorcluster, "Collection out"=w308:refnum<class "Collection.lvclass">)  [unwired: 7 in]
        n124 = property class="Line.lvclass"(reference=refnum<class "Line.lvclass"> refnum ("LvMarkdown.lvlib:Line.lvclass"), "Text"="and here's a longer one.") -> (reference out=w318:refnum<class "Line.lvclass">)  [unwired: 1 in, 1 out]
        n125 = property class="Line.lvclass"(reference=refnum<class "Line.lvclass"> refnum ("LvMarkdown.lvlib:Line.lvclass"), "Text"="Here's a simple footnote,") -> (reference out=w333:refnum<class "Line.lvclass">)  [unwired: 1 in, 1 out]
        n126 = property class="Footnote.lvclass"(reference=refnum<class "Footnote.lvclass"> refnum ("LvMarkdown.lvlib:Footnote.lvclass"), "FootnoteReference"=w314, "Text"="Here's one with multiple paragraphs and code.\n\nIndent paragraphs to include them in the footnote.\n\n`{ my code }`\n\nAdd as many paragraphs as you like.") -> (reference out=w312:refnum<class "Footnote.lvclass">)  [unwired: 1 in, 1 out]
        n127 = property class="Footnote.lvclass"(reference=refnum<class "Footnote.lvclass"> refnum ("LvMarkdown.lvlib:Footnote.lvclass"), "FootnoteReference"=w321, "Text"="This is the first footnote.") -> (reference out=w313:refnum<class "Footnote.lvclass">)  [unwired: 1 in, 1 out]
        n128 = call-dynamic "AddToCollection.vi"("error in (no error)"=w310, "IRenderable"=w333, "Collection in"=w308) -> ("error out"=w331:errorcluster, "Collection out"=w332:refnum<class "Collection.lvclass">)  [unwired: 7 in]
        n129 = call-dynamic "AddToCollection.vi"("error in (no error)"=w331, "IRenderable"=w321, "Collection in"=w332) -> ("error out"=w329:errorcluster, "Collection out"=w330:refnum<class "Collection.lvclass">)  [unwired: 7 in]
        n130 = call-dynamic "AddToCollection.vi"("error in (no error)"=w329, "IRenderable"=w318, "Collection in"=w330) -> ("error out"=w327:errorcluster, "Collection out"=w328:refnum<class "Collection.lvclass">)  [unwired: 7 in]
        n131 = call-dynamic "AddToCollection.vi"("error in (no error)"=w327, "IRenderable"=w314, "Collection in"=w328) -> ("error out"=w326:errorcluster, "Collection out"=w306:refnum<class "Collection.lvclass">)  [unwired: 7 in]
        n132 = call-dynamic "AddToCollection.vi"("error in (no error)"=w326, "IRenderable"=w304, "Collection in"=w306) -> ("error out"=w307:errorcluster, "Collection out"=w305:refnum<class "Collection.lvclass">)  [unwired: 7 in]
        n133 = call-dynamic "AddToCollection.vi"("error in (no error)"=w307, "IRenderable"=w313, "Collection in"=w305) -> ("error out"=w324:errorcluster, "Collection out"=w325:refnum<class "Collection.lvclass">)  [unwired: 7 in]
        n134 = call-dynamic "AddToCollection.vi"("error in (no error)"=w324, "IRenderable"=w312, "Collection in"=w325) -> ("error out"=w323:errorcluster, "Collection out"=w322:refnum<class "Collection.lvclass">)  [unwired: 7 in]
      }
      frame "LinkingHeadingId" {
        n135 = property class="LinkingHeadingId.lvclass"(reference=refnum<class "LinkingHeadingId.lvclass"> refnum ("LvMarkdown.lvlib:LinkingHeadingId.lvclass"), "Text"="Link to Heading 2", "Heading"=w340) -> (reference out=w347:refnum<class "LinkingHeadingId.lvclass">)  [unwired: 1 in, 1 out]
        n136 = call-dynamic "AddToCollection.vi"("error in (no error)"=w342, "IRenderable"=w341, "Collection in"=w343) -> ("error out"=w345:errorcluster, "Collection out"=w348:refnum<class "Collection.lvclass">)  [unwired: 7 in]
        n137 = call-dynamic "AddToCollection.vi"("error in (no error)"=w345, "IRenderable"=w347, "Collection in"=w348) -> ("error out"=w344:errorcluster, "Collection out"=w346:refnum<class "Collection.lvclass">)  [unwired: 7 in]
      }
      frame "DefinitionList" {
        n138 = Build Array("This is one definition of the second term." ("Definition"), "This is another definition of the second term." ("Definition")) -> (w360:string[])
        n139 = Build Array("This is the definition of the first term." ("Definition")) -> (w361:string[])
        n140 = property class="DefinitionList.lvclass"(reference=refnum<class "DefinitionList.lvclass"> refnum ("LvMarkdown.lvlib:DefinitionList.lvclass"), "Term"="Second Term", "Definitions"=w360) -> (reference out=w352:refnum<class "DefinitionList.lvclass">)  [unwired: 1 in, 1 out]
        n141 = property class="DefinitionList.lvclass"(reference=refnum<class "DefinitionList.lvclass"> refnum ("LvMarkdown.lvlib:DefinitionList.lvclass"), "Term"="First Term", "Definitions"=w361) -> (reference out=w365:refnum<class "DefinitionList.lvclass">)  [unwired: 1 in, 1 out]
        n142 = call-dynamic "AddToCollection.vi"("error in (no error)"=w364, "IRenderable"=w365, "Collection in"=w367) -> ("error out"=w355:errorcluster, "Collection out"=w356:refnum<class "Collection.lvclass">)  [unwired: 7 in]
        n143 = call-dynamic "AddToCollection.vi"("error in (no error)"=w355, "IRenderable"=w352, "Collection in"=w356) -> ("error out"=w354:errorcluster, "Collection out"=w353:refnum<class "Collection.lvclass">)  [unwired: 7 in]
      }
      frame "Exit" {
        n144 = Current VI's Path() -> (path=w376:path)
        n145 = Strip Path(path=w376) -> (stripped path=w375:path)  [unwired: 1 out]
        n146 = call-dynamic "Render.vi"("error in (no error)"=w368, "String in"="", "Collection in"=w372) -> ("error out"=w370:errorcluster, "String out"=→"String out":string, "Collection out"=w377:refnum<class "Collection.lvclass">)  [unwired: 6 in]
        n147 = Build Path(base path=w375, name or relative path=path "../docs/Test.md") -> (appended path=w374:path)
        n148 = call "Save.vi"("error in (no error)"=w370, "Path"=w374, "Collection in"=w377) -> ("error out"=w369:errorcluster, "Collection out"=w371:refnum<class "Collection.lvclass">)  [unwired: 7 in]
      }
    }
  }
